vi "VIH ProjFile - HHP Generation - Convert Paths.vi"(5 "Build Root Dir":path, 7 "Project Dir":path, 10 "Operation":enum16{"Read", "Write"}(ring), 11 "HHP_Generation":T1={"HHP_Template"=enum."default", "HHP_Template_CustomPath"=path "", "HHP_Target"=enum."default", "HHP_Target_CustomPath"=path "", "HHP_CreateTOC"=TRUE, "HHP_CreateIDX"=TRUE, "HHP_DefaultTopic"=enum."auto", "HHP_DefaultTopic_CustomPath"=path "", "CHM_Filename"=path "", "HHP_AutoBuild"=FALSE, "CHM_AutoBuild"=FALSE}) -> (3 "HHP_Generation out":T1={"HHP_Template"=enum."default", "HHP_Template_CustomPath"=path "", "HHP_Target"=enum."default", "HHP_Target_CustomPath"=path "", "HHP_CreateTOC"=TRUE, "HHP_CreateIDX"=TRUE, "HHP_DefaultTopic"=enum."auto", "HHP_DefaultTopic_CustomPath"=path "", "CHM_Filename"=path "", "HHP_AutoBuild"=FALSE, "CHM_AutoBuild"=FALSE})   [LabVIEW 2014]
doc: "::: VI Helpeks :::\nCopyright (c) 2000-2026 Konstantin Shifershteyn. All rights reserved."
uses:
  _VIH CHM Project.llb/VIH - CHM Project - HHP Generation Params Cluster.ctl
panel:
  # "VI Helpeks\nCopyright (c) 2012-2026 Konstantin Shifershteyn"
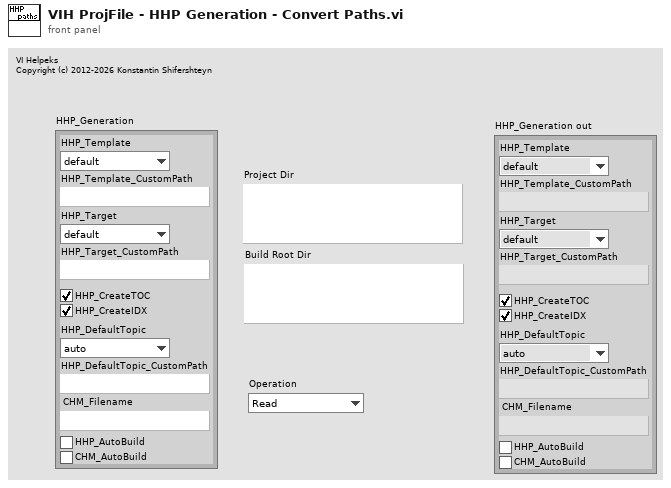
[diagram p1: front panel]
types:
  T1 = typedef "VIH - CHM Project - HHP Generation Params Cluster.ctl" = cluster{"HHP_Template":enum16{"default", "custom"}, "HHP_Template_CustomPath":path, "HHP_Target":enum16{"default", "custom"}, "HHP_Target_CustomPath":path, "HHP_CreateTOC":bool, "HHP_CreateIDX":bool, "HHP_DefaultTopic":enum16{"auto", "custom"}, "HHP_DefaultTopic_CustomPath":path, "CHM_Filename":path, "HHP_AutoBuild":bool, "CHM_AutoBuild":bool}
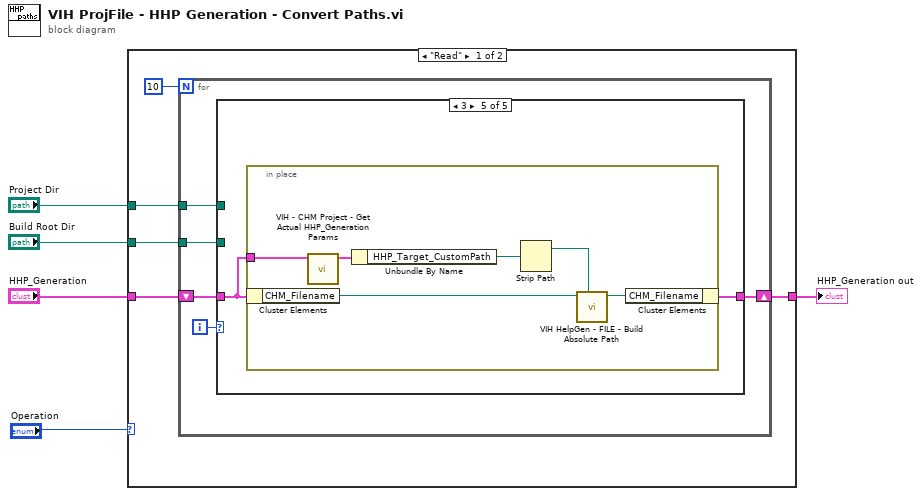
[diagram p0: block diagram]
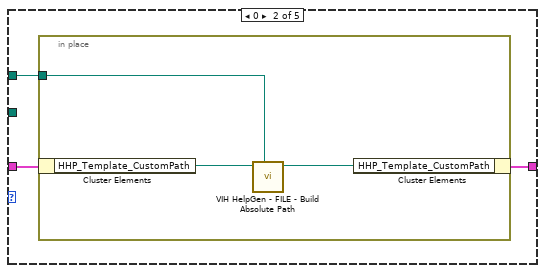
[diagram p3: hidden frame]
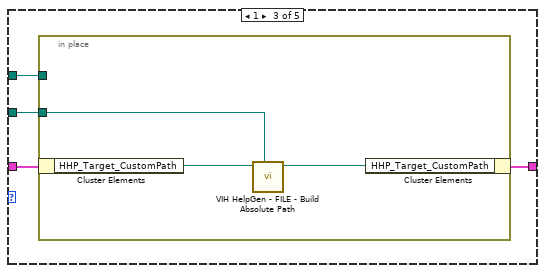
[diagram p4: hidden frame]
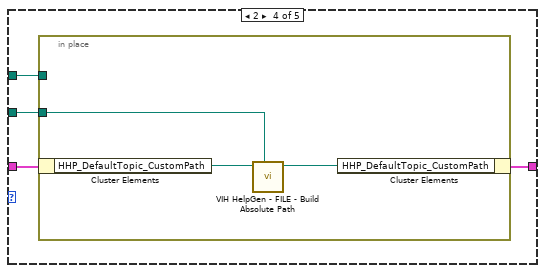
[diagram p5: hidden frame]
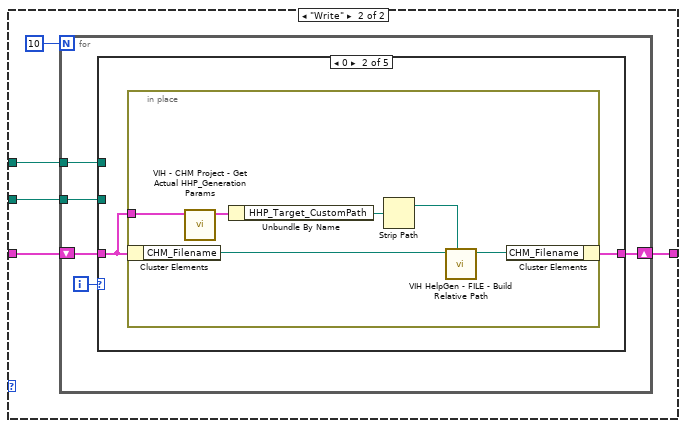
[diagram p6: hidden frame]
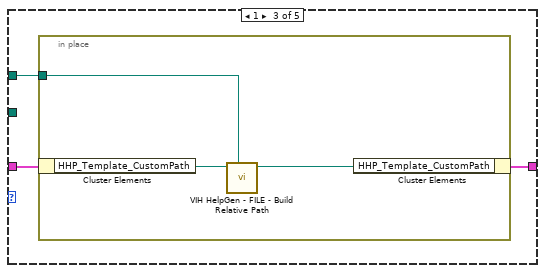
[diagram p8: hidden frame]
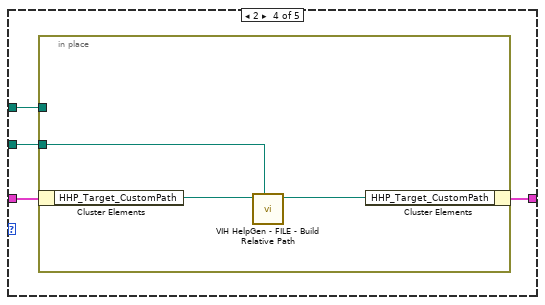
[diagram p9: hidden frame]
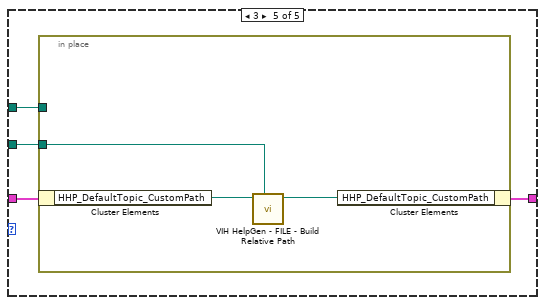
[diagram p10: hidden frame]
diagram:
  n1 = case shown="\"Read\"" "Operation" {
    tunnel: "Project Dir" -> [w9 w48]
    tunnel: "HHP_Generation" -> [w8 w47]
    tunnel: [w7 w46] -> w2
    tunnel: "Build Root Dir" -> [w6 w45]
    frame "Read" {
      n2 = for {
        N: 10 -> [_]
        tunnel: w9 -> [w14]
        shift-right: [w12] -> w7
        shift-left: w8 -> [w13]
        tunnel: w6 -> [w11]
        i -> [w15]
        n3 = case shown="3" w15 {
          tunnel: w14 -> [_ w19 w26 w33 _]
          tunnel: w13 -> [w16 w18 w25 w32 w37]
          tunnel: [w16 w17 w24 w31 w38] -> w12
          tunnel: w11 -> [_ _ w23 w30 _]
          frame Default {
          }
          frame 0 {
            n4 = in-place {
              in-place-border: w19 -> [w21]
              n5 = in-place-cluster #1(w18) -> ("HHP_Template_CustomPath"=w22:path)
              n6 = call "VIH HelpGen - FILE - Build Absolute Path.vi"("Root Path"=w21, "Path in"=w22) -> ("Path out"=w20:path)  [unwired: 9 in]
              n7 = in-place-cluster #1("HHP_Template_CustomPath"=w20) -> (w17:T1)
            }
          }
          frame 1 {
            n8 = in-place {
              in-place-border: w26 -> [_]
              in-place-border: w23 -> [w27]
              n9 = in-place-cluster #2(w25) -> ("HHP_Target_CustomPath"=w29:path)
              n10 = call "VIH HelpGen - FILE - Build Absolute Path.vi"("Root Path"=w27, "Path in"=w29) -> ("Path out"=w28:path)  [unwired: 9 in]
              n11 = in-place-cluster #2("HHP_Target_CustomPath"=w28) -> (w24:T1)
            }
          }
          frame 2 {
            n12 = in-place {
              in-place-border: w33 -> [_]
              in-place-border: w30 -> [w34]
              n13 = in-place-cluster #3(w32) -> ("HHP_DefaultTopic_CustomPath"=w36:path)
              n14 = call "VIH HelpGen - FILE - Build Absolute Path.vi"("Root Path"=w34, "Path in"=w36) -> ("Path out"=w35:path)  [unwired: 9 in]
              n15 = in-place-cluster #3("HHP_DefaultTopic_CustomPath"=w35) -> (w31:T1)
            }
          }
          frame 3 {
            n16 = in-place {
              in-place-border: w37 -> [w41]
              n17 = in-place-cluster #4(w37) -> ("CHM_Filename"=w44:path)
              n18 = call "VIH - CHM Project - Get Actual HHP_Generation Params.vi"("HHP_Generation"=w41) -> ("HHP_Generation out"=w42:T1)  [unwired: 8 in, 2 out]
              n19 = Unbundle By Name(w42) -> ("HHP_Target_CustomPath"=w40:path)
              n20 = Strip Path(path=w40) -> (stripped path=w39:path)  [unwired: 1 out]
              n21 = call "VIH HelpGen - FILE - Build Absolute Path.vi"("Root Path"=w39, "Path in"=w44) -> ("Path out"=w43:path)  [unwired: 9 in]
              n22 = in-place-cluster #4("CHM_Filename"=w43) -> (w38:T1)
            }
          }
        }
      }
    }
    frame "Write" {
      n23 = for {
        N: 10 -> [_]
        tunnel: w48 -> [w53]
        shift-right: [w51] -> w46
        shift-left: w47 -> [w52]
        tunnel: w45 -> [w50]
        i -> [w54]
        n24 = case shown="0" w54 {
          tunnel: w53 -> [_ _ w66 w73 w80]
          tunnel: w52 -> [w55 w56 w65 w72 w79]
          tunnel: [w55 w57 w64 w71 w78] -> w51
          tunnel: w50 -> [_ _ _ w70 w77]
          frame Default {
          }
          frame 0 {
            n25 = in-place {
              in-place-border: w56 -> [w60]
              n26 = in-place-cluster #5(w56) -> ("CHM_Filename"=w63:path)
              n27 = call "VIH - CHM Project - Get Actual HHP_Generation Params.vi"("HHP_Generation"=w60) -> ("HHP_Generation out"=w61:T1)  [unwired: 8 in, 2 out]
              n28 = Unbundle By Name(w61) -> ("HHP_Target_CustomPath"=w59:path)
              n29 = Strip Path(path=w59) -> (stripped path=w58:path)  [unwired: 1 out]
              n30 = call "VIH HelpGen - FILE - Build Relative Path.vi"("Root Path"=w58, "Path in"=w63) -> ("Path out"=w62:path)  [unwired: 9 in]
              n31 = in-place-cluster #5("CHM_Filename"=w62) -> (w57:T1)
            }
          }
          frame 1 {
            n32 = in-place {
              in-place-border: w66 -> [w67]
              n33 = in-place-cluster #6(w65) -> ("HHP_Template_CustomPath"=w69:path)
              n34 = call "VIH HelpGen - FILE - Build Relative Path.vi"("Root Path"=w67, "Path in"=w69) -> ("Path out"=w68:path)  [unwired: 9 in]
              n35 = in-place-cluster #6("HHP_Template_CustomPath"=w68) -> (w64:T1)
            }
          }
          frame 2 {
            n36 = in-place {
              in-place-border: w73 -> [_]
              in-place-border: w70 -> [w74]
              n37 = in-place-cluster #7(w72) -> ("HHP_Target_CustomPath"=w76:path)
              n38 = call "VIH HelpGen - FILE - Build Relative Path.vi"("Root Path"=w74, "Path in"=w76) -> ("Path out"=w75:path)  [unwired: 9 in]
              n39 = in-place-cluster #7("HHP_Target_CustomPath"=w75) -> (w71:T1)
            }
          }
          frame 3 {
            n40 = in-place {
              in-place-border: w80 -> [_]
              in-place-border: w77 -> [w81]
              n41 = in-place-cluster #8(w79) -> ("HHP_DefaultTopic_CustomPath"=w83:path)
              n42 = call "VIH HelpGen - FILE - Build Relative Path.vi"("Root Path"=w81, "Path in"=w83) -> ("Path out"=w82:path)  [unwired: 9 in]
              n43 = in-place-cluster #8("HHP_DefaultTopic_CustomPath"=w82) -> (w78:T1)
            }
          }
        }
      }
    }
  }
  "HHP_Generation out" <- w2
